vi "Rebuild tree.vi"(8 "error in":errorcluster, 10 "Headers":string[](array[string]), 11 "References":T1) -> (0 "error out":errorcluster)   [LabVIEW 2025, in "CAN-LIN Raw Bus Capture UI.lvlib"]
uses:
  CAN-LIN Raw Bus Capture UI.lvlib
panel:
  out "Value":string[][](array[string])
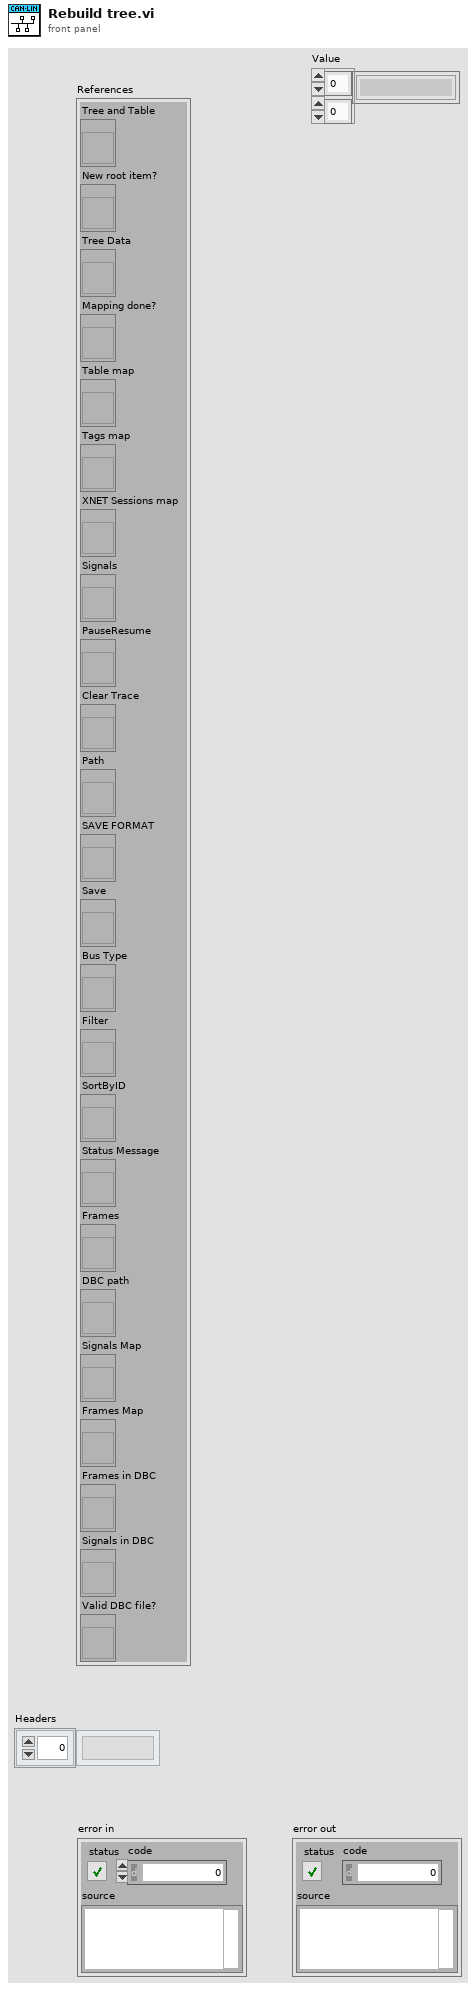
[diagram p1: front panel]
types:
  T1 = cluster{"Tree and Table":refnum<vi>, "New root item?":refnum<vi>, "Tree Data":refnum<vi>, "Mapping done?":refnum<vi>, "Table map":refnum<vi>, "Tags map":refnum<vi>, "XNET Sessions map":refnum<vi>, "Signals":refnum<vi>, "PauseResume":refnum<vi>, "Clear Trace":refnum<vi>, "Path":refnum<vi>, "SAVE FORMAT":refnum<vi>, "Save":refnum<vi>, "Bus Type":refnum<vi>, "Filter":refnum<vi>, "SortByID":refnum<vi>, "Status Message":refnum<vi>, "Frames":refnum<vi>, "DBC path":refnum<vi>, "Signals Map":refnum<vi>, "Frames Map":refnum<vi>, "Frames in DBC":refnum<vi>, "Signals in DBC":refnum<vi>, "Valid DBC file?":refnum<vi>}
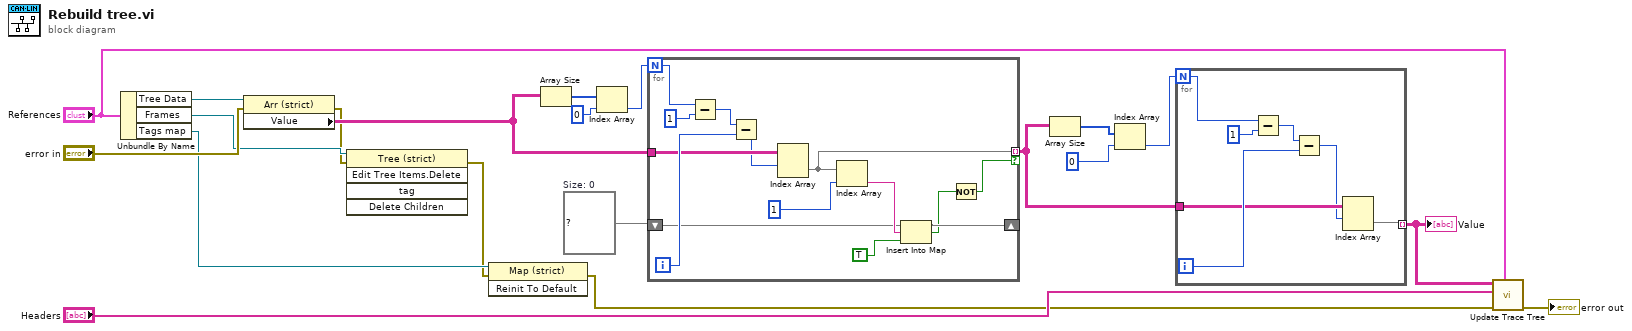
[diagram p0: block diagram]
diagram:
  w15 = map{string, bool} {}  # Size: 0
  n1 = Unbundle By Name("References") -> ("Tree Data"=w20:refnum<vi>, "Frames"=w9:refnum<vi>, "Tags map"=w7:refnum<vi>)
  n2 = property class="Arr (strict)"(reference=w20, error in="error in") -> (error out=w8:errorcluster, "Value"=w19:string[][])  [unwired: 1 out]
  n3 = invoke class="Tree (strict)" method="Edit Tree Items.Delete"(reference=w9, error in=w8) -> (error out=w6:errorcluster)  [unwired: 3 in, 4 out]
  n4 = invoke class="Map (strict)" method="Reinit To Default"(reference=w7, error in=w6) -> (error out=w2:errorcluster)  [unwired: 1 in, 2 out]
  n5 = Array Size(array=w19) -> (size(s)=w18:i32[])
  n6 = Index Array(array=w18, index=0) -> (element=w16:i32)
  n7 = for {
    N: w16 -> [w33]
    tunnel: w19 -> [w30]
    shift-right: [w25] -> _
    shift-left: w15 -> [w24]
    tunnel: [w23] -> w11 mode=indexing if=w21
    i -> [w31]
    n8 = Subtract(x=w33, y=1) -> (x-y=w32:i32)
    n9 = Subtract(x=w32, y=w31) -> (x-y=w29:i32)
    n10 = Index Array(array=w30, index (row)=w29) -> (element=w23:string[])  [unwired: 1 in]
    n11 = Index Array(array=w23, index=1) -> (element=w27:string)
    n12 = Insert Into Map(map in=w24, key=w27, value=TRUE) -> (map out=w25:map{string, bool}, key already included?=w22:bool)  [unwired: 1 out]
    n13 = Not(x=w22) -> (.not. x?=w21:bool)
  }
  n14 = Array Size(array=w11) -> (size(s)=w14:i32[])
  n15 = Index Array(array=w14, index=0) -> (element=w12:i32)
  n16 = for {
    N: w12 -> [w39]
    tunnel: w11 -> [w37]
    tunnel: [w35] -> w5 mode=indexing
    i -> [w38]
    n17 = Subtract(x=w39, y=1) -> (x-y=w40:i32)
    n18 = Subtract(x=w40, y=w38) -> (x-y=w36:i32)
    n19 = Index Array(array=w37, index (row)=w36) -> (element=w35:string[])  [unwired: 1 in]
  }
  "Value" <- w5
  n20 = call "Update Trace Tree.vi"("References"="References", "error in"=w2, "Headers"="Headers", "Data IN"=w5) -> ("error out"=→"error out":errorcluster)  [unwired: 6 in, 1 out]
